vi "Get ControlRef from ClassItem.vi"(8 "error in (no error)":errorcluster, 10 "item name":string, 11 "class in":refnum<vi>) -> (0 "error out":errorcluster, 1 "control":refnum<vi>, 2 "VI ref out":refnum<vi>, 3 "class out":refnum<vi>, 4 "found":bool)   [LabVIEW 2019, in "gRPC Template Creation Utility.lvlib"]
uses:
  gRPC Template Creation Utility.lvlib
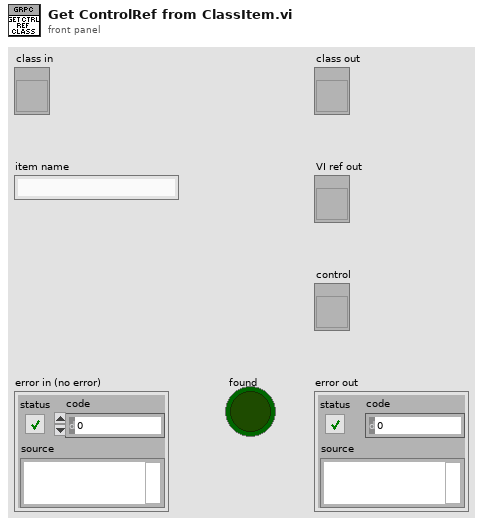
[diagram p1: front panel]
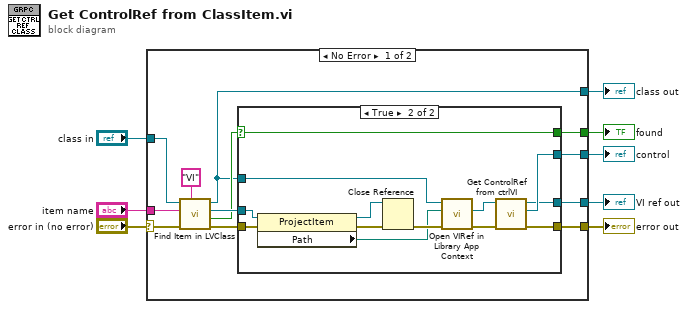
[diagram p0: block diagram]
diagram:
  n1 = case shown="No Error" "error in (no error)" {
    selector: "error in (no error)" -> [w13 w36]
    tunnel: [w20 _] -> w8
    tunnel: "class in" -> [w17 w37]
    tunnel: "item name" -> [w15 _]
    tunnel: [w10 w37] -> w5
    tunnel: [w14 w36] -> w4
    tunnel: [w11 _] -> w2
    tunnel: [w9 _] -> w1
    frame No Error {
      n2 = call "Find Item in LVClass.vi"("Item Type"="VI", "error in (no error)"=w13, "Item Name"=w15, "Class Item in"=w17) -> ("error out"=w19:errorcluster, "Found?"=w12:bool, "Project Item (Class Item)"=w18:refnum<vi>, "Class Item out"=w10:refnum<vi>)  [unwired: 4 in]
      n3 = case shown="True" w12 {
        selector: w12 -> [w21 w32]
        tunnel: [_ w35] -> w20
        tunnel: w19 -> [w22 w34]
        tunnel: w18 -> [_ w33]
        tunnel: [w22 w29] -> w14
        tunnel: [w21 w32] -> w11
        tunnel: w10 -> [_ w23]
        tunnel: [_ w28] -> w9
        frame False {
        }
        frame True {
          n4 = property class="ProjectItem"(reference=w33, error in=w34) -> (reference out=w30:refnum<vi>, error out=w31:errorcluster, "Path"=w25:path)
          n5 = Close Reference(reference=w30, error in (no error)=w31) -> (error out=w26:errorcluster)
          n6 = call "Open VIRef in Library App Context.vi"("error in (no error)"=w26, "vi path"=w25, "library in"=w23) -> ("error out"=w27:errorcluster, "vi"=w24:refnum<vi>)  [unwired: 6 in, 1 out]
          n7 = call "Get ControlRef from ctrlVI.vi"("error in (no error)"=w27, "VI ref in"=w24) -> ("error out"=w29:errorcluster, "Control ref out"=w35:refnum<vi>, "VI ref out"=w28:refnum<vi>)  [unwired: 7 in]
        }
      }
    }
    frame Error {
    }
  }
  "control" <- w8
  "class out" <- w5
  "error out" <- w4
  "found" <- w2
  "VI ref out" <- w1
